vi "Check For item.vi"(8 "This Name":string, 9 "short names":string[](array[string]), 10 "item paths":path[](array[path]), 11 "This Path":path) -> (0 "index of element":i32, 1 "Flattened Name":string, 2 "Short Name":string)   [LabVIEW 2012, in "Palette Generation.lvlib"]
doc: "Attempts to locate an item for possible inclusion ina palette based on (1) whether it's short name matches an existing short name and (2) whether it's path matches an existing palette item path.\n\nThis avoids having two shortnames that are identical but with different paths which appears to be an illegal palette definition"
uses:
  Palette Generation.lvlib
  <userlib>/_OpenG.lib/file/file.llb/Strip Path - Traditional__ogtk.vi
  <vilib>/regexp/Match Regular Expression.xnode
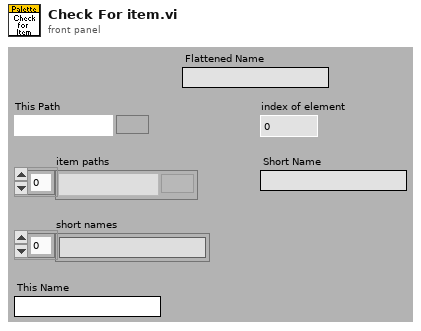
[diagram p1: front panel]
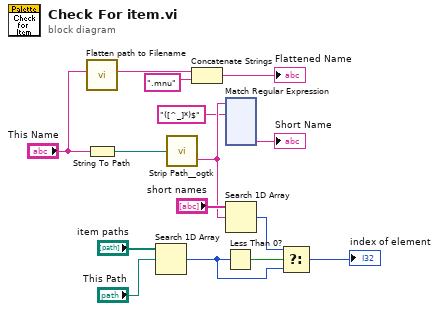
[diagram p0: block diagram]
diagram:
  n1 = call "Flatten path to Filename.vi"("Virtual Folder's Virtual Path"="This Name") -> ("result string"=w6:string)  [unwired: 2 in, 7 out]
  n2 = String To Path(string="This Name") -> (path=w10:path)
  n3 = Search 1D Array(1D array="item paths", element="This Path") -> (index of element=w15:i32)  [unwired: 1 out]
  n4 = call-poly <userlib>:"Strip Path__ogtk.vi"("path"=w10) -> ("name"=w3:string)  [unwired: 1 out]
  n5 = Concatenate Strings(w6, ".mnu" ("string")) -> (→"Flattened Name":string)
  n6 = Less Than 0?(x=w15) -> (x < 0?=w13:bool)
  n7 = xnode "Match Regular Expression"("input string"=w3, "regular expression"="([^_]*)$") -> ("submatch 1"=→"Short Name":string)  [unwired: 2 in, 7 out]
  n8 = Search 1D Array(1D array="short names", element=w3) -> (index of element=w14:i32)  [unwired: 1 in]
  n9 = Select(t=w14, s=w13, f=w15) -> (s? t:f=→"index of element":i32)
